vi "UE_Retry_Allowed.vi"(1 "max_attempts":i32, 2 "attempts_used":i32) -> (0 "allowed":bool)   [LabVIEW 2026]
doc: "INTENT: True if retry attempts used is lower than configured maximum. INPUTS: attempts_used (int32), max_attempts (int32). OUTPUTS: allowed (bool). DESIGN CONSTRAINT: Attempt counting semantics must be consistent with scheduler. REQUIREMENTS: SRS-F-010. No physical hardware side effects. Acceptance requires native LabVIEW compilation and behavioral testing."
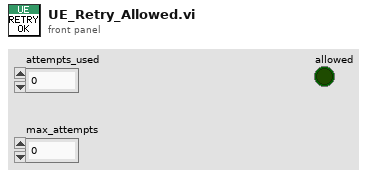
[diagram p1: front panel]
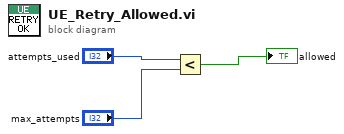
[diagram p0: block diagram]
diagram:
  n1 = Less?(x="attempts_used", y="max_attempts") -> (x < y?=→"allowed":bool)
